vi "AlliGator with Detachable Panels Register Control Events.vi"(8 "Error In":errorcluster) -> (0 "Error Out":errorcluster, 3 "AlliGator Events Registration":T1)   [LabVIEW 2021, in "AlliGator GUI.lvlib"]
doc: "Registers user events for controls on the main AlliGator window."
uses:
  AlliGator GUI.lvlib
  AlliGator with Detachable Panels Events Registration.ctl
  Settings/AlliGator Settings Event.ctl
  Settings/AlliGator Settings Window Messages.ctl
  Phasor Plot Color Map/AlliGator Phasor Color Map User Event List.ctl
  AlliGator Subpanel Event Data.ctl
  Settings/AlliGator Settings+.lvlib
  Phasor Plot Color Map/AlliGator Phasor Plot Color Map.lvlib
panel:
  # "see the AlliGator License on the block diagram (Ctrl+E or Window:Show Block Diagram)"
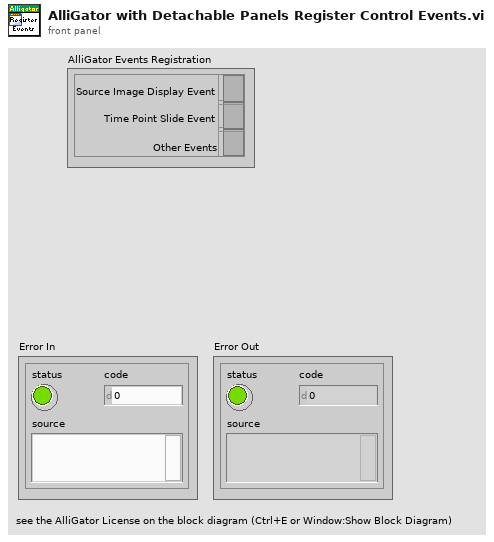
[diagram p1: front panel]
types:
  T1 = typedef "AlliGator GUI.lvlib/AlliGator with Detachable Panels Events Registration.ctl" = cluster{"Source Image Display Event":refnum<event-registration>, "Time Point Slide Event":refnum<event-registration>, "Other Events":refnum<event-registration>}
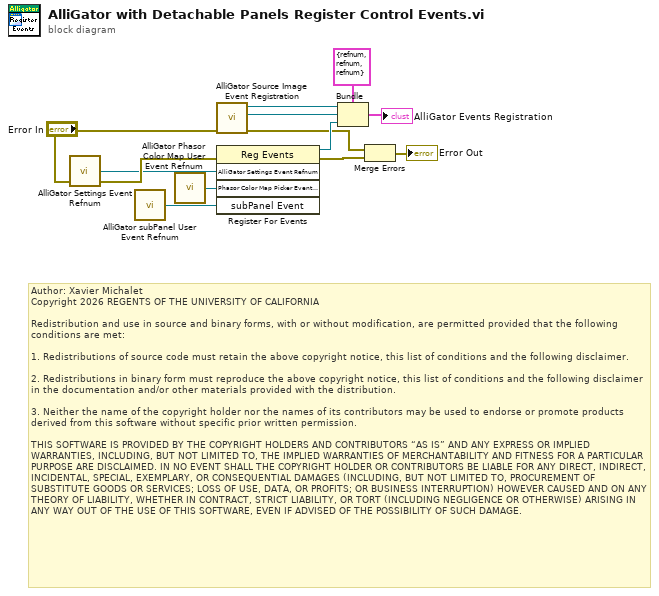
[diagram p0: block diagram]
diagram:
  # "Author: Xavier Michalet\nCopyright 2026 REGENTS OF THE UNIVERSITY OF CALIFORNIA\n\nRedistribution and use in source and binary forms, with or without modification, are permitted provided that the following conditions are met:\n\n1. Redistributions of source code must retain the above copyright notice, this list of conditions and the following disclaimer.\n\n2. Redistributions in binary form must reproduce the above copyright notice, this list of conditions and the following disclaimer in the documentation and/or other materials provided with the distribution.\n\n3. Neither the name of the copyright holder nor the names of its contributors may be used to endorse or promote products derived from this software without specific prior written permission.\n\nTHIS SOFTWARE IS PROVIDED BY THE COPYRIGHT HOLDERS AND CONTRIBUTORS “AS IS” AND ANY EXPRESS OR IMPLIED WARRANTIES, INCLUDING, BUT NOT LIMITED TO, THE IMPLIED WARRANTIES OF MERCHANTABILITY AND FITNESS FOR A PARTICULAR PURPOSE ARE DISCLAIMED. IN NO EVENT SHALL THE COPYRIGHT HOLDER OR CONTRIBUTORS BE LIABLE FOR ANY DIRECT, INDIRECT, INCIDENTAL, SPECIAL, EXEMPLARY, OR CONSEQUENTIAL DAMAGES (INCLUDING, BUT NOT LIMITED TO, PROCUREMENT OF SUBSTITUTE GOODS OR SERVICES; LOSS OF USE, DATA, OR PROFITS; OR BUSINESS INTERRUPTION) HOWEVER CAUSED AND ON ANY THEORY OF LIABILITY, WHETHER IN CONTRACT, STRICT LIABILITY, OR TORT (INCLUDING NEGLIGENCE OR OTHERWISE) ARISING IN ANY WAY OUT OF THE USE OF THIS SOFTWARE, EVEN IF ADVISED OF THE POSSIBILITY OF SUCH DAMAGE."
  n1 = call "AlliGator Settings Event Refnum.vi"("Error In"="Error In") -> ("AlliGator Settings Event Refnum"=w5:refnum<user-event>, "Error Out"=w6:errorcluster)  [unwired: 7 in]
  n2 = call "AlliGator subPanel User Event Refnum.vi"() -> ("subPanel Event"=w10:refnum<user-event>)  [unwired: 9 in]
  n3 = call "AlliGator Phasor Color Map User Event Refnum.vi"() -> ("Phasor Color Map Picker Event Refnum"=w11:refnum<user-event>)  [unwired: 9 in]
  n4 = call "AlliGator Source Image Event Registration.vi"("error in (no error)"="Error In") -> ("error out"=w3:errorcluster, "Time Point Slide Event Registration"=w7:refnum<event-registration>, "Source Image Display Event Registration"=w12:refnum<event-registration>)  [unwired: 8 in]
  n5 = register-events(error in=w6, w5, w11, w10) -> (reference out=w9:refnum<event-registration>, error out=w8:errorcluster)  [unwired: 1 in]
  n6 = Bundle(cluster=T1 {"Source Image Display Event"=refnum, "Time Point Slide Event"=refnum, "Other Events"=refnum} ("AlliGator Events Registration"), "Source Image Display Event"=w12, "Time Point Slide Event"=w7, "Other Events"=w9) -> (→"AlliGator Events Registration":T1)
  n7 = Merge Errors(w3, w8) -> (→"Error Out":errorcluster)
